vi "Build.vi"(6 "ItemBuilt":T1, 8 "error in (no error)":errorcluster, 11 "BuildManager in":refnum<class "BuildManager.lvclass">) -> (0 "error out":errorcluster, 3 "BuildManager out":refnum<class "BuildManager.lvclass">)   [LabVIEW 2019, in "SolutionBuilder.lvlib" / "BuildManager.lvclass"]
uses:
  BuildManager.lvclass
  Events/EventItemBuilt.ctl
  BuildManager.lvclass/BuildManager.ctl
  ProjectItem/ProjectItem.lvclass
  SolutionBuilder.lvlib
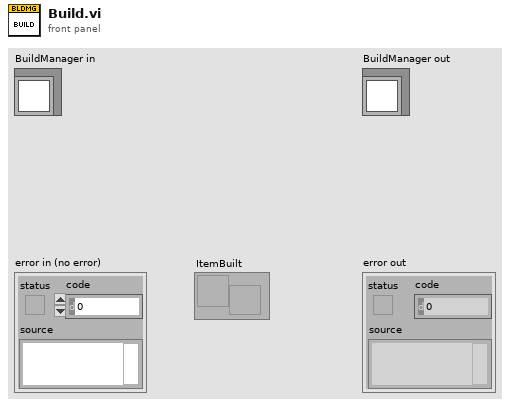
[diagram p1: front panel]
types:
  T1 = typedef "SolutionBuilder.lvlib/EventItemBuilt.ctl" = refnum<user-event>
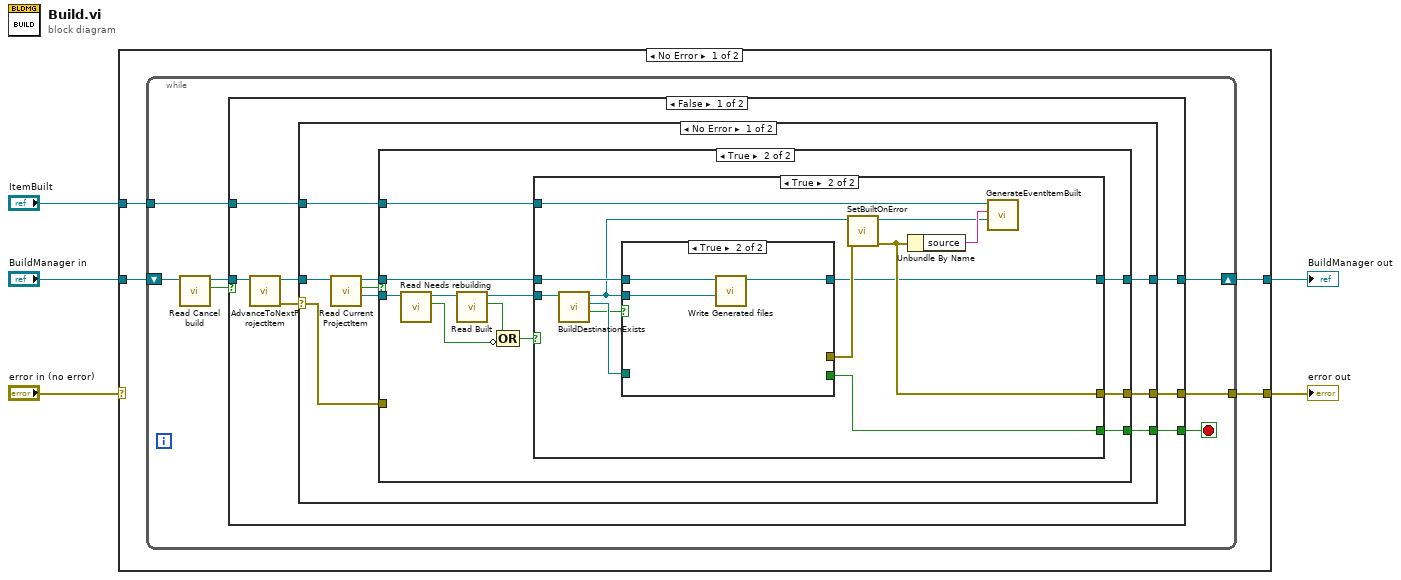
[diagram p0: block diagram]
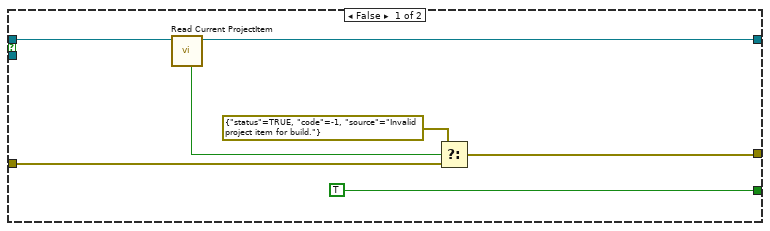
[diagram p2: hidden frame]
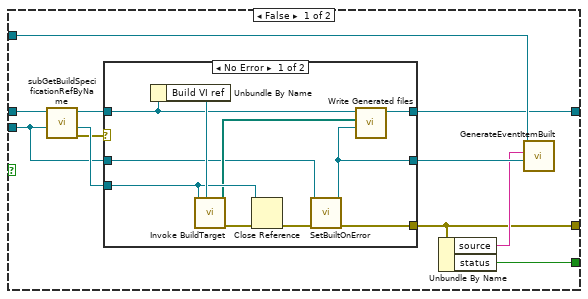
[diagram p3: hidden frame]
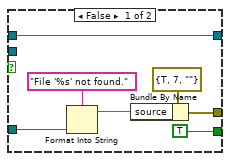
[diagram p5: hidden frame]
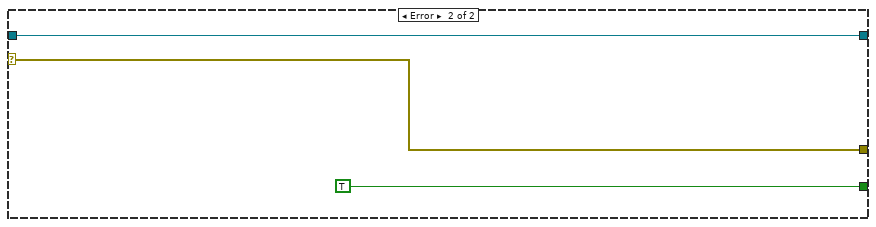
[diagram p6: hidden frame]
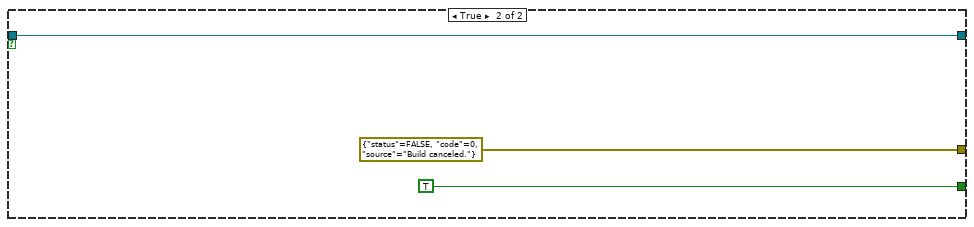
[diagram p7: hidden frame]
diagram:
  n1 = case shown="No Error" "error in (no error)" {
    selector: "error in (no error)" -> [_ w104]
    tunnel: "BuildManager in" -> [w9 w103]
    tunnel: "ItemBuilt" -> [w8 _]
    tunnel: [w6 w104] -> w2
    tunnel: [w7 w103] -> w1
    frame No Error {
      n2 = while {
        shift-right: [w16] -> w7
        shift-left: w9 -> [w12]
        tunnel: w8 -> [w14]
        tunnel: [w13] -> w6
        stop <- w15 stop-if-true
        n3 = call "Read Cancel build.vi"("BuildManager in"=w12) -> ("Cancel?"=w10:bool, "BuildManager out"=w11:refnum<class "BuildManager.lvclass">)  [unwired: 9 in]
        n4 = case shown="False" w10 {
          tunnel: [w22 w102] -> w16
          tunnel: [w21 TRUE] -> w15
          tunnel: w14 -> [w20 _]
          tunnel: [w19 errorcluster {"status"=FALSE, "code"=0, "source"="Build canceled."} ("t")] -> w13
          tunnel: w11 -> [w17 w102]
          frame False {
            n5 = call "AdvanceToNextProjectItem.vi"("BuildManager in"=w17) -> ("error out"=w18:errorcluster, "BuildManager out"=w23:refnum<class "BuildManager.lvclass">)  [unwired: 9 in]
            n6 = case shown="No Error" w18 {
              selector: w18 -> [w24 w97]
              tunnel: w23 -> [w32 w99]
              tunnel: [w28 w99] -> w22
              tunnel: [w27 TRUE ("status")] -> w21
              tunnel: w20 -> [w26 _]
              tunnel: [w25 w97] -> w19
              frame No Error {
                n7 = call "Read Current ProjectItem.vi"("BuildManager in"=w32) -> ("Current ProjectItem"=w29:refnum<class "ProjectItem.lvclass">, "Valid"=w31:bool, "BuildManager out"=w30:refnum<class "BuildManager.lvclass">)  [unwired: 7 in, 1 out]
                n8 = case shown="True" w31 {
                  tunnel: w30 -> [w37 w50]
                  tunnel: w29 -> [_ w43]
                  tunnel: [w38 w49] -> w28
                  tunnel: [TRUE w46] -> w27
                  tunnel: w26 -> [_ w47]
                  tunnel: [w33 w45] -> w25
                  tunnel: w24 -> [w34 _]
                  frame False {
                    n9 = call "Read Current ProjectItem.vi"("BuildManager in"=w37) -> ("BuildManager out"=w38:refnum<class "BuildManager.lvclass">, "In bounds"=w36:bool)  [unwired: 7 in, 2 out]
                    n10 = Select(t=errorcluster {"status"=TRUE, "code"=-1, "source"="Invalid project item for build."}, s=w36, f=w34) -> (s? t:f=w33:errorcluster)
                  }
                  frame True {
                    n11 = call "Read Needs rebuilding.vi"("ProjectItem in"=w43) -> ("Needs rebuilding"=w41:bool, "ProjectItem out"=w44:refnum<class "ProjectItem.lvclass">)  [unwired: 9 in]
                    n12 = call "Read Built.vi"("ProjectItem in"=w44) -> ("Built"=w42:bool, "ProjectItem out"=w48:refnum<class "ProjectItem.lvclass">)  [unwired: 9 in]
                    n13 = Compound Arithmetic op=OR(w42, invert w41) -> (w40:bool)
                    n14 = case shown="True" w40 {
                      tunnel: w50 -> [w61 w80]
                      tunnel: [w54 w79] -> w49
                      tunnel: w48 -> [w51 w78]
                      tunnel: w47 -> [w58 w83]
                      tunnel: [w56 w86] -> w46
                      tunnel: [w52 w84] -> w45
                      frame False {
                        n15 = call "subGetBuildSpecificationRefByName.vi"("ProjectItem in"=w51, "BuildManager in"=w61) -> ("error out"=w53:errorcluster, "Build spec ref"=w60:refnum<vi>, "BuildManager out"=w55:refnum<class "BuildManager.lvclass">)  [unwired: 7 in]
                        n16 = case shown="No Error" w53 {
                          selector: w53 -> [_ w72]
                          tunnel: w60 -> [w69 _]
                          tunnel: w51 -> [w63 w73]
                          tunnel: [w62 w73] -> w59
                          tunnel: [w70 w72] -> w52
                          tunnel: w55 -> [w65 w74]
                          tunnel: [w66 w74] -> w54
                          frame No Error {
                            n17 = Unbundle By Name(w65) -> ("Build VI ref"=w71:refnum<vi>)
                            n18 = call <vilib>:"Invoke BuildTarget.vi"("vi reference"=w71, "BuildItem ref"=w69) -> ("error out"=w68:errorcluster, "Generated files"=w64:path[])  [unwired: 8 in]
                            n19 = Close Reference(reference=w69, error in (no error)=w68) -> (error out=w67:errorcluster)
                            n20 = call "SetBuiltOnError.vi"("error in (no error)"=w67, "ProjectItem in"=w63) -> ("error out"=w70:errorcluster, "ProjectItem out"=w62:refnum<class "ProjectItem.lvclass">)  [unwired: 8 in]
                            n21 = call "Write Generated files.vi"("ProjectItem in"=w62, "Generated files"=w64, "BuildManager in"=w65) -> ("BuildManager out"=w66:refnum<class "BuildManager.lvclass">)  [unwired: 8 in]
                          }
                          frame Error {
                          }
                        }
                        n22 = Unbundle By Name(w52) -> ("source"=w57:string, "status"=w56:bool)
                        n23 = call "GenerateEventItemBuilt.vi"("ProjectItem"=w59, "Result"=w57, "ItemBuilt"=w58) -> ()  [unwired: 9 in]
                      }
                      frame True {
                        n24 = call "BuildDestinationExists.vi"("ProjectItem in"=w78) -> ("Exists"=w75:bool, "path out"=w76:path, "ProjectItem out"=w77:refnum<class "ProjectItem.lvclass">)  [unwired: 7 in, 1 out]
                        n25 = case shown="True" w75 {
                          tunnel: [w90 _] -> w85
                          tunnel: w76 -> [w89 _]
                          tunnel: [TRUE _] -> w86
                          tunnel: w80 -> [w87 w96]
                          tunnel: [w87 w95] -> w79
                          tunnel: w77 -> [_ w94]
                          frame False {
                            n26 = Format Into String(format string="File '%s' not found.", w89) -> (resulting string=w91:string)  [unwired: 2 in, 1 out]
                            n27 = Bundle By Name(cluster=errorcluster {"status"=TRUE, "code"=7, "source"=""} ("error out"), "source"=w91) -> (w90:errorcluster)
                          }
                          frame True {
                            n28 = call "Write Generated files.vi"("ProjectItem in"=w94, "BuildManager in"=w96) -> ("BuildManager out"=w95:refnum<class "BuildManager.lvclass">)  [unwired: 9 in]
                          }
                        }
                        n29 = call "SetBuiltOnError.vi"("error in (no error)"=w85, "ProjectItem in"=w77) -> ("error out"=w84:errorcluster, "ProjectItem out"=w81:refnum<class "ProjectItem.lvclass">)  [unwired: 8 in]
                        n30 = Unbundle By Name(w84) -> ("source"=w82:string)
                        n31 = call "GenerateEventItemBuilt.vi"("ProjectItem"=w81, "Result"=w82, "ItemBuilt"=w83) -> ()  [unwired: 9 in]
                      }
                    }
                  }
                }
              }
              frame Error {
              }
            }
          }
          frame True {
          }
        }
      }
    }
    frame Error {
    }
  }
  "error out" <- w2
  "BuildManager out" <- w1
